vi "Update.vi"(8 "error in (no error)":errorcluster, 10 "Audio Data In":dbl[][](array[numeric]), 11 "Flanger in":refnum<class "Flanger.lvclass">) -> (0 "error out":errorcluster, 2 "Audio Data Out":dbl[][](array[numeric]), 3 "Flanger out":refnum<class "Flanger.lvclass">)   [LabVIEW 2019, in "Flanger.lvlib" / "Flanger.lvclass"]
doc: "Applies the flanger effect. The effect is produced by adding a duplicate audio signal to the original, with a slowly shifting phase.\n\n<b>Value1:</b> Dry/wet amount\n<b>Value2:</b> Phase shift frequency"
uses:
  Flanger.lvclass
  Flanger.lvclass/Flanger.ctl
  <vilib>/ptbypt/NI_PtbyPt.lvlib
  Plugin Interfaces/Effect Interface/Effect Interface.lvlibp/Effect Interface Class/Effect Interface.lvclass
  C:/github/dataflowg/dataflow-dj/src/Plugin Interfaces/Effect Interface/Effect Interface.lvlibp/Plugin Interfaces/Effect Interface/Effect Interface Class/Effect Interface.lvclass
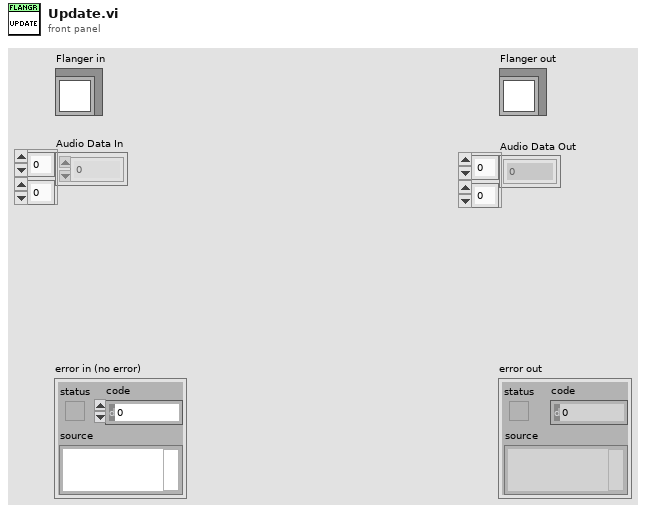
[diagram p1: front panel]
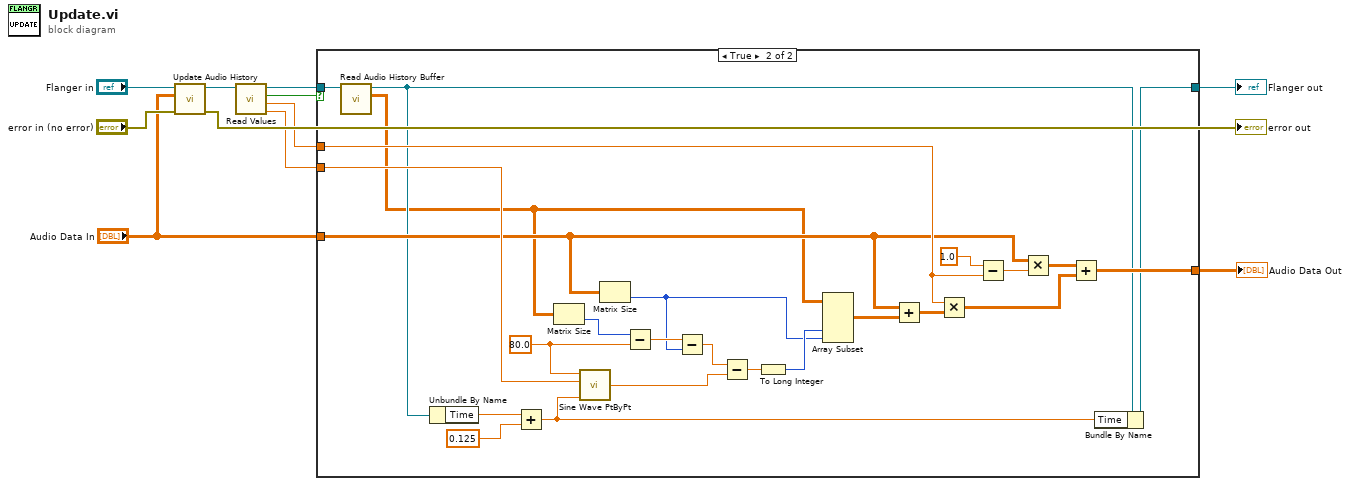
[diagram p0: block diagram]
diagram:
  n1 = call "Update Audio History.vi"("error in (no error)"="error in (no error)", "Audio Data In"="Audio Data In", "Effect Interface in"="Flanger in") -> ("error out"=→"error out":errorcluster, "Effect Interface out"=w6:refnum<class "Flanger.lvclass">)  [unwired: 7 in]
  n2 = call "Read Values.vi"("Effect Interface in"=w6) -> ("Value2"=w1:dbl, "Value1"=w3:dbl, "Enable"=w2:bool, "Effect Interface out"=w5:refnum<class "Flanger.lvclass">)  [unwired: 7 in]
  n3 = case shown="True" w2 {
    tunnel: w3 -> [_ w23]
    tunnel: w1 -> [_ w22]
    tunnel: [w12 w21] -> w11
    tunnel: [w13 w19] -> w10
    tunnel: "Audio Data In" -> [w12 w17]
    tunnel: w5 -> [w13 w14]
    frame False {
    }
    frame True {
      w29 = 80.0 ("Delay")
      n4 = call "Read Audio History Buffer.vi"("Effect Interface in"=w14) -> ("Audio History Buffer"=w15:dbl[][], "Effect Interface out"=w16:refnum<class "Flanger.lvclass">)  [unwired: 9 in]
      n5 = Unbundle By Name(w16) -> ("Time"=w20:dbl)
      n6 = Add(x=w20, y=0.125) -> (x+y=w18:dbl)
      n7 = Matrix Size(0:w15) -> (2:w24:i32)  [unwired: 1 out]
      n8 = call <vilib>:"Sine Wave PtByPt.vi"("time"=w18, "frequency"=w22, "amplitude"=w29) -> ("sine wave"=w26:dbl)  [unwired: 1 in]
      n9 = Matrix Size(0:w17) -> (2:w25:i32)  [unwired: 1 out]
      n10 = Subtract(x=w24, y=w29) -> (x-y=w30:dbl)
      n11 = Subtract(x=w30, y=w25) -> (x-y=w31:dbl)
      n12 = Subtract(x=w31, y=w26) -> (x-y=w27:dbl)
      n13 = To Long Integer(number=w27) -> (32bit integer=w28:i32)
      n14 = Array Subset(array=w15, index (col)=w28, length (col)=w25) -> (w38:dbl[][])  [unwired: 2 in]
      n15 = Add(x=w17, y=w38) -> (x+y=w33:dbl[][])
      n16 = Multiply(x=w23, y=w33) -> (x*y=w37:dbl[][])
      n17 = Subtract(x=1.0, y=w23) -> (x-y=w35:dbl)
      n18 = Multiply(x=w17, y=w35) -> (x*y=w36:dbl[][])
      n19 = Add(x=w36, y=w37) -> (x+y=w21:dbl[][])
      n20 = Bundle By Name(cluster=w16, "Time"=w18) -> (w19:refnum<class "Flanger.lvclass">)
    }
  }
  "Audio Data Out" <- w11
  "Flanger out" <- w10
